vi "Tag.vi"(0 "obj in":refnum<class "Sensor.lvclass">) -> (1 "tag":string)   [LabVIEW 2026, in "Sensor.lvclass"]
doc: "Round15 P15: Sensor's own dynamic method returning a class tag string. obj in is a path stand-in retyped to Sensor with dynamic dispatch by lvai_add_class_method; the diagram ignores the object and returns a constant."
uses:
  Sensor.lvclass
  Sensor.lvclass/Sensor.ctl
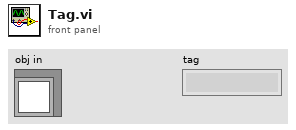
[diagram p1: front panel]
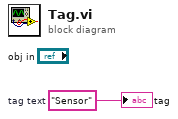
[diagram p0: block diagram]
diagram:
  w1 = "Sensor"  # tag text
  "tag" <- w1
